vi "Test U8 Change FIFO Size.vi"() -> ()   [LabVIEW 2021]
uses:
  ChannelCommon/typedef/Direction.ctl
  ChannelCommon/typedef/TimeStamps.ctl
  CIF_Iceoryx_PCAP_Universal.lvclass
  D:/dev/Packages/CIF_Channels_Core/src/Iceorxy_Channels/CIF_Iceoryx_Chan/CIF_Iceoryx_Chn.lvclass
  ChannelCommon/typedef/New FIFO Instance Configuration.ctl
  Iceorxy Utilities/Typedef/PCAP Config.ctl
  ChannelCommon/typedef/New FIFO Config.ctl
  ChannelCommon/typedef/FIFO Flags.ctl
  Iceorxy Utilities/Typedef/PCAP Linktype.ctl
  CIF_Iceoryx_Chan/CIF_Iceoryx_Chn.lvclass
  ChannelCommon/ChannelCommon.lvlib
  Iceorxy Utilities/Iceoryx Channel Utilities.lvlib
panel:
  out "status":string
  out "pass":bool
  out "error out":errorcluster
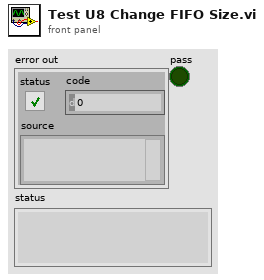
[diagram p1: front panel]
types:
  T1 = typedef "ChannelCommon.lvlib/Direction.ctl" = enum8{"Publisher", "Subscriber"}
  T2 = typedef "Iceoryx Channel Utilities.lvlib/PCAP Config.ctl" = cluster{"New FIFO Config":T3, "Linktype":T5, "Linktype Override":u32, "Type Name Override":string}
  T3 = typedef "ChannelCommon.lvlib/New FIFO Config.ctl" = cluster{"Max Bytes/Msg":u64, "Max Msg/FIFO":u64, "FIFO Flags":T4, "Best Effort Subscribers":u32, "Backpressure Subscribers":u32}
  T4 = typedef "ChannelCommon.lvlib/FIFO Flags.ctl" = cluster{"Backpressure":bool, "Extended Config":bool}
  T5 = typedef "Iceoryx Channel Utilities.lvlib/PCAP Linktype.ctl" = u32
  T6 = typedef "ChannelCommon.lvlib/New FIFO Instance Configuration.ctl" = cluster{"Backpressure":bool, "Bytes/Message Override":u32, "Messages/FIFO Override":u32, "Custom Data":u8[]}
  T7 = typedef "ChannelCommon.lvlib/TimeStamps.ctl" = cluster{"ClockID":u8, "T0":i64, "T_Out":i64}
  T8 = typedef "ChannelCommon.lvlib/New FIFO Instance Response.ctl" = cluster{"Publisher":string, "Custom Data":u8[]}
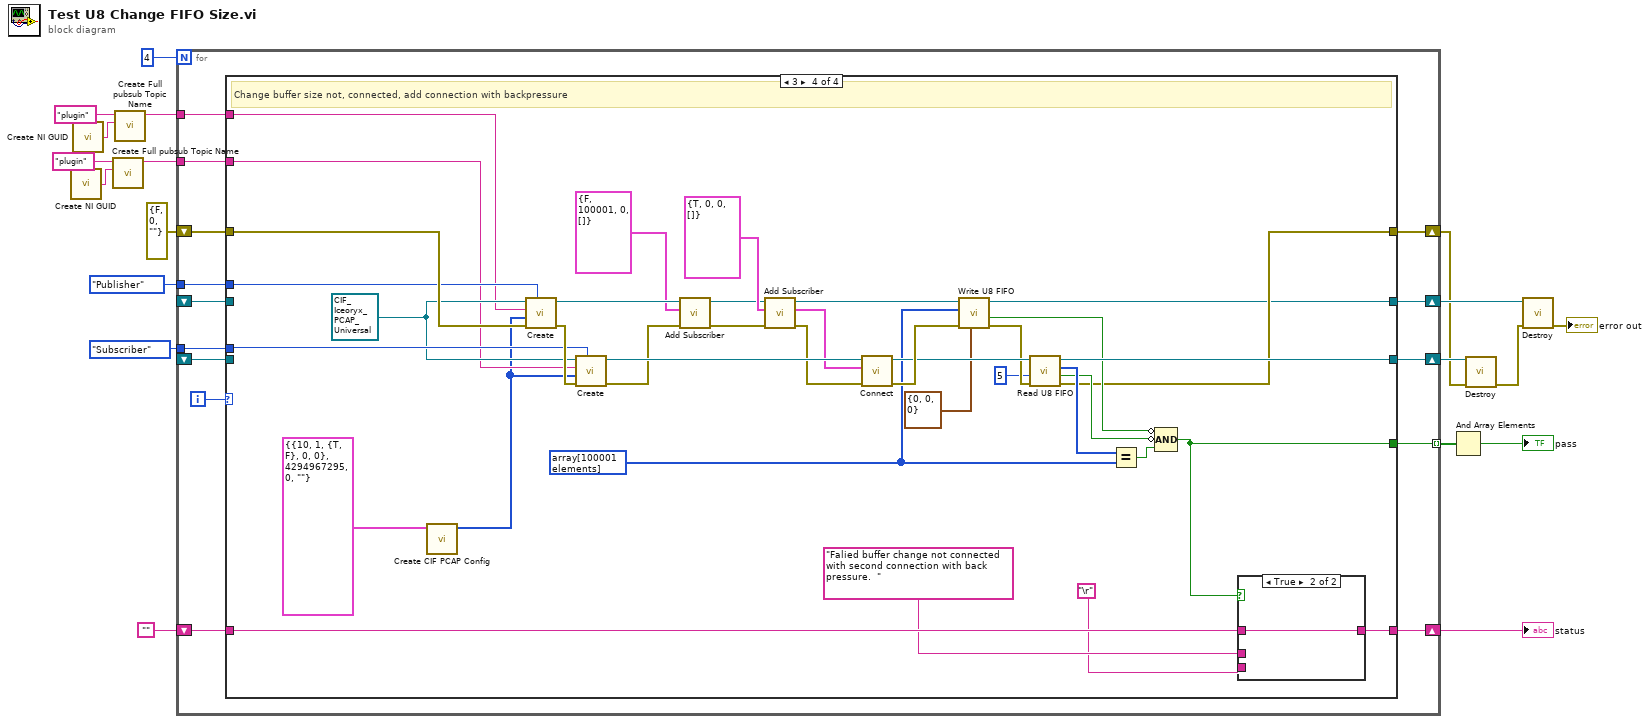
[diagram p0: block diagram]
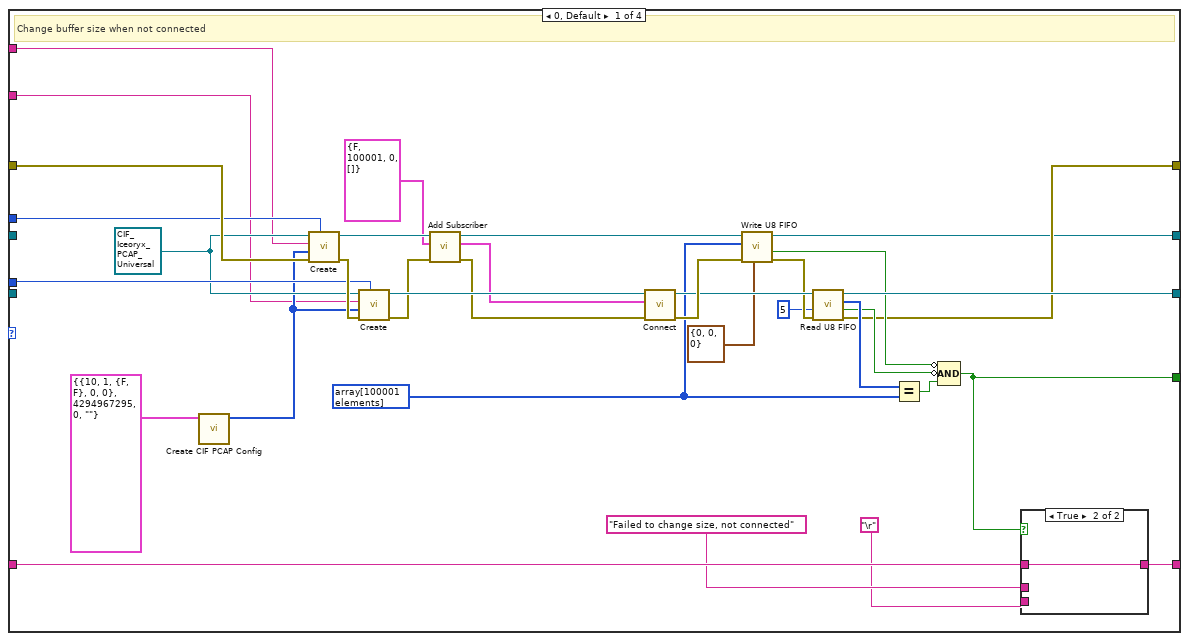
[diagram p2: hidden frame]
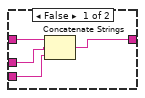
[diagram p3: hidden frame]
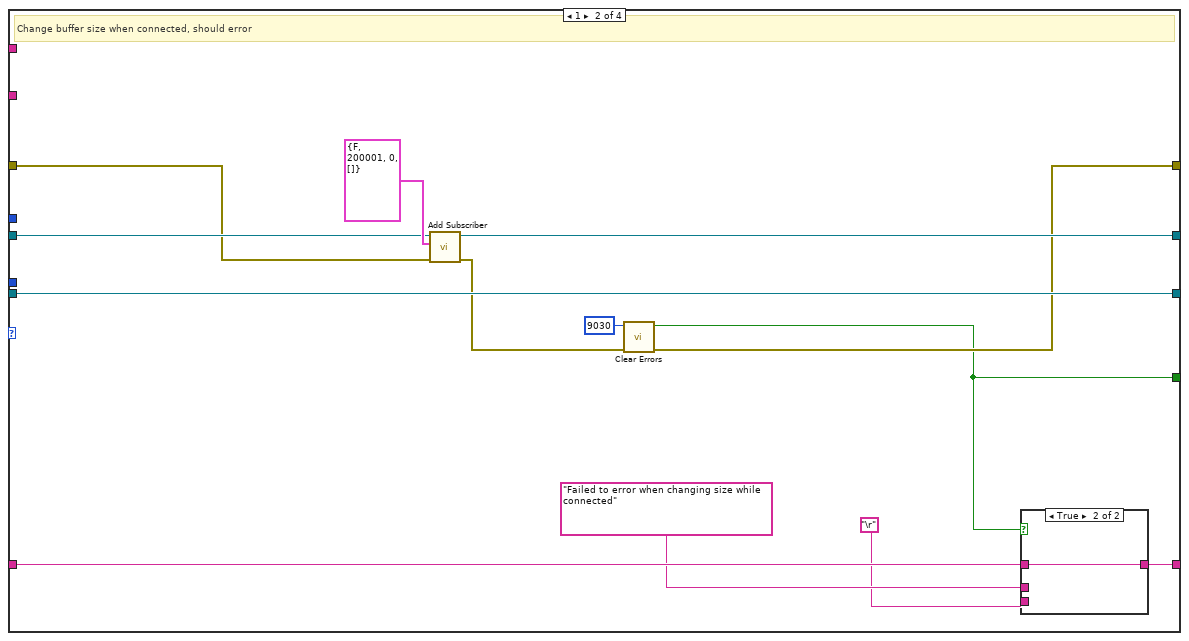
[diagram p4: hidden frame]
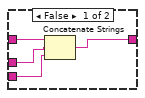
[diagram p5: hidden frame]
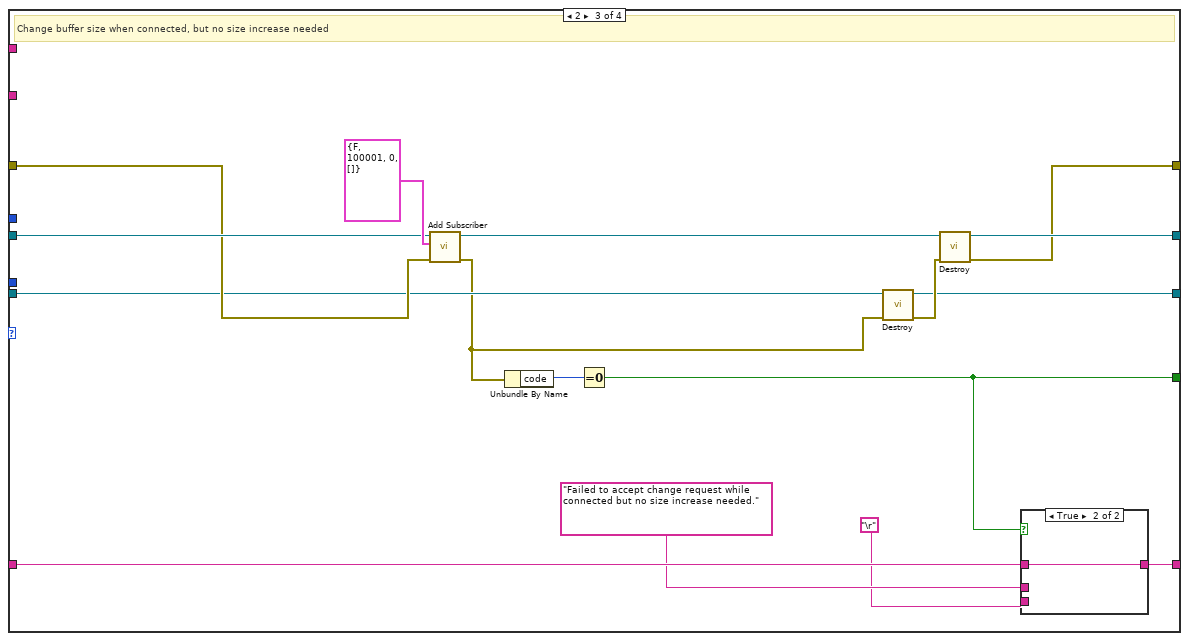
[diagram p6: hidden frame]
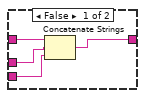
[diagram p7: hidden frame]
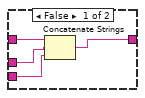
[diagram p8: hidden frame]
diagram:
  n1 = call <vilib>:"Create NI GUID.vi"() -> ("NI GUID"=w6:string)
  n2 = call <vilib>:"Create NI GUID.vi"() -> ("NI GUID"=w5:string)
  n3 = call "Create Full pubsub Topic Name.vi"("Topic"=w6, "Plugin name"="plugin") -> ("Full Topic"=w2:string)  [unwired: 8 in, 1 out]
  n4 = call "Create Full pubsub Topic Name.vi"("Topic"=w5, "Plugin name"="plugin") -> ("Full Topic"=w1:string)  [unwired: 8 in, 1 out]
  n5 = for {
    N: 4 -> [_]
    tunnel: [w33] -> w19 mode=indexing
    shift-right: [w31] -> w8
    shift-left: errorcluster {"status"=FALSE, "code"=0, "source"=""} ("error out") -> [w32]
    shift-right: [w28] -> w15
    shift-left: "" -> [w29]
    tunnel: Direction."Subscriber" ("Direction") -> [w27]
    tunnel: Direction."Publisher" ("Direction") -> [w26]
    shift-right: [w25] -> w11
    shift-left: _ -> [w23]
    shift-right: [w24] -> w10
    shift-left: _ -> [w22]
    tunnel: w2 -> [w21]
    tunnel: w1 -> [w20]
    i -> [w30]
    n6 = case shown="3" w30 {
      tunnel: [w62 w73 w98 w143] -> w33
      tunnel: w32 -> [w60 w79 w100 w141]
      tunnel: [w45 w75 w91 w126] -> w31
      tunnel: w29 -> [w67 w85 w106 w148]
      tunnel: [w66 w84 w105 w147] -> w28
      tunnel: w27 -> [w59 _ _ w140]
      tunnel: w26 -> [w58 _ _ w139]
      tunnel: [w54 w78 w92 w135] -> w25
      tunnel: [w44 w77 w93 w125] -> w24
      tunnel: w22 -> [_ w80 w101 _]
      tunnel: w23 -> [_ w78 w96 _]
      tunnel: w21 -> [w35 _ _ w114]
      tunnel: w20 -> [w34 _ _ w115]
      frame 0, Default {
        w49 = refnum<class "CIF_Iceoryx_PCAP_Universal.lvclass"> refnum ("CIF_CIPC_Fifo_U8.lvclass")
        w46 = u8[] array[100001 elements] ("U8 Data")
        # "Change buffer size when not connected"
        n7 = call "Create CIF PCAP Config.vi"("PCAP FIFO Config"=T2 {"New FIFO Config"={"Max Bytes/Msg"=10, "Max Msg/FIFO"=1, "FIFO Flags"={"Backpressure"=FALSE, "Extended Config"=FALSE}, "Best Effort Subscribers"=0, "Backpressure Subscribers"=0}, "Linktype"=4294967295, "Linktype Override"=0, "Type Name Override"=""}) -> ("Flattened PCAP FIFO Config"=w36:u8[])  [unwired: 10 in]
        n8 = call-dynamic "Create.vi"("Direction"=w58, "error in (no error)"=w60, "Custom Config Data"=w36, "Name"=w34, "CIFFIFO in"=w49) -> ("error out"=w61:errorcluster, "CIFFIFO out"=w43:refnum<class "CIF_Iceoryx_PCAP_Universal.lvclass">)  [unwired: 5 in]
        n9 = call-dynamic "Create.vi"("Direction"=w59, "error in (no error)"=w61, "Custom Config Data"=w36, "Name"=w35, "CIFFIFO in"=w49) -> ("error out"=w39:errorcluster, "CIFFIFO out"=w57:refnum<class "CIF_Iceoryx_PCAP_Universal.lvclass">)  [unwired: 5 in]
        n10 = call-dynamic "Add Subscriber.vi"("error in (no error)"=w39, "New FIFO Instance Config"=T6 {"Backpressure"=FALSE, "Bytes/Message Override"=100001, "Messages/FIFO Override"=0, "Custom Data"=[]}, "CIF_CIPC_Chn in"=w43) -> ("error out"=w38:errorcluster, "New FIFO Instance"=w41:T8, "CIF_CIPC_Chn out"=w42:refnum<class "CIF_Iceoryx_PCAP_Universal.lvclass">)  [unwired: 6 in]
        n11 = call-dynamic "Connect.vi"("error in (no error)"=w38, "Connection"=w41, "CIF_Iceoryx_PCAP"=w57) -> ("error out"=w56:errorcluster, "CIF_Iceoryx_PCAP"=w55:refnum<class "CIF_Iceoryx_PCAP_Universal.lvclass">)  [unwired: 7 in]
        n12 = call-dynamic "Write U8 FIFO.vi"("FIFO Timestamps"=T7 {"ClockID"=0, "T0"=0, "T_Out"=0}, "error in (no error)"=w56, "Data in"=w46, "CIFFIFO in"=w42) -> ("error out"=w53:errorcluster, "timed out?"=w52:bool, "CIFFIFO out"=w44:refnum<class "CIF_Iceoryx_PCAP_Universal.lvclass">)  [unwired: 4 in, 1 out]
        n13 = call-dynamic "Read U8 FIFO.vi"("error in (no error)"=w53, "Timeout (ms)"=5, "CIFFIFO in"=w55) -> ("error out"=w45:errorcluster, "timed out?"=w50:bool, "Data out"=w51:u8[], "CIFFIFO out"=w54:refnum<class "CIF_Iceoryx_PCAP_Universal.lvclass">)  [unwired: 4 in, 1 out]
        n14 = Equal?(x=w51, y=w46) -> (x = y?=w63:bool)
        n15 = Compound Arithmetic op=AND(invert w52, invert w50, w63) -> (w62:bool)
        n16 = case shown="True" w62 {
          tunnel: w67 -> [w71 w72]
          tunnel: [w68 w72] -> w66
          tunnel: "Failed to change size, not connected" -> [w70 _]
          tunnel: "\r" -> [w69 _]
          frame False {
            n17 = Concatenate Strings(w71, w70, w69) -> (w68:string)
          }
          frame True {
          }
        }
      }
      frame 1 {
        # "Change buffer size when connected, should error"
        n18 = call-dynamic "Add Subscriber.vi"("error in (no error)"=w79, "New FIFO Instance Config"=T6 {"Backpressure"=FALSE, "Bytes/Message Override"=200001, "Messages/FIFO Override"=0, "Custom Data"=[]}, "CIF_CIPC_Chn in"=w80) -> ("error out"=w76:errorcluster, "CIF_CIPC_Chn out"=w77:refnum<class "CIF_Iceoryx_Chn.lvclass">)  [unwired: 6 in, 1 out]
        n19 = call <vilib>:"Clear Errors.vi"("error in (no error)"=w76, "specific error code to clear (0: all)"=9030) -> ("error out"=w75:errorcluster, "specific error cleared?"=w73:bool)  [unwired: 4 in]
        n20 = case shown="True" w73 {
          tunnel: w85 -> [w89 w90]
          tunnel: [w86 w90] -> w84
          tunnel: "Failed to error when changing size while connected" -> [w88 _]
          tunnel: "\r" -> [w87 _]
          frame False {
            n21 = Concatenate Strings(w89, w88, w87) -> (w86:string)
          }
          frame True {
          }
        }
      }
      frame 2 {
        # "Change buffer size when connected, but no size increase needed"
        n22 = call-dynamic "Add Subscriber.vi"("error in (no error)"=w100, "New FIFO Instance Config"=T6 {"Backpressure"=FALSE, "Bytes/Message Override"=100001, "Messages/FIFO Override"=0, "Custom Data"=[]}, "CIF_CIPC_Chn in"=w101) -> ("error out"=w94:errorcluster, "CIF_CIPC_Chn out"=w95:refnum<class "CIF_Iceoryx_Chn.lvclass">)  [unwired: 6 in, 1 out]
        n23 = Unbundle By Name(w94) -> ("code"=w99:i32)
        n24 = Equal To 0?(x=w99) -> (x = 0?=w98:bool)
        n25 = call-dynamic "Destroy.vi"("error in (no error)"=w94, "CIFChannels in"=w96) -> ("error out"=w97:errorcluster, "CIFChannels out"=w92:refnum<class "CIF_Iceoryx_Chn.lvclass">)  [unwired: 8 in]
        n26 = call-dynamic "Destroy.vi"("error in (no error)"=w97, "CIFChannels in"=w95) -> ("error out"=w91:errorcluster, "CIFChannels out"=w93:refnum<class "CIF_Iceoryx_Chn.lvclass">)  [unwired: 8 in]
        n27 = case shown="True" w98 {
          tunnel: w106 -> [w110 w111]
          tunnel: [w107 w111] -> w105
          tunnel: "Failed to accept change request while connected but no size increase needed." -> [w109 _]
          tunnel: "\r" -> [w108 _]
          frame False {
            n28 = Concatenate Strings(w110, w109, w108) -> (w107:string)
          }
          frame True {
          }
        }
      }
      frame 3 {
        w130 = refnum<class "CIF_Iceoryx_PCAP_Universal.lvclass"> refnum ("CIF_CIPC_Fifo_U8.lvclass")
        w127 = u8[] array[100001 elements] ("U8 Data")
        # "Change buffer size not, connected, add connection with backpressure"
        n29 = call "Create CIF PCAP Config.vi"("PCAP FIFO Config"=T2 {"New FIFO Config"={"Max Bytes/Msg"=10, "Max Msg/FIFO"=1, "FIFO Flags"={"Backpressure"=TRUE, "Extended Config"=FALSE}, "Best Effort Subscribers"=0, "Backpressure Subscribers"=0}, "Linktype"=4294967295, "Linktype Override"=0, "Type Name Override"=""}) -> ("Flattened PCAP FIFO Config"=w112:u8[])  [unwired: 10 in]
        n30 = call-dynamic "Create.vi"("Direction"=w139, "error in (no error)"=w141, "Custom Config Data"=w112, "Name"=w115, "CIFFIFO in"=w130) -> ("error out"=w142:errorcluster, "CIFFIFO out"=w120:refnum<class "CIF_Iceoryx_PCAP_Universal.lvclass">)  [unwired: 5 in]
        n31 = call-dynamic "Create.vi"("Direction"=w140, "error in (no error)"=w142, "Custom Config Data"=w112, "Name"=w114, "CIFFIFO in"=w130) -> ("error out"=w117:errorcluster, "CIFFIFO out"=w138:refnum<class "CIF_Iceoryx_PCAP_Universal.lvclass">)  [unwired: 5 in]
        n32 = call-dynamic "Add Subscriber.vi"("error in (no error)"=w117, "New FIFO Instance Config"=T6 {"Backpressure"=FALSE, "Bytes/Message Override"=100001, "Messages/FIFO Override"=0, "Custom Data"=[]}, "CIF_CIPC_Chn in"=w120) -> ("error out"=w118:errorcluster, "CIF_CIPC_Chn out"=w119:refnum<class "CIF_Iceoryx_PCAP_Universal.lvclass">)  [unwired: 6 in, 1 out]
        n33 = call-dynamic "Add Subscriber.vi"("error in (no error)"=w118, "New FIFO Instance Config"=T6 {"Backpressure"=TRUE, "Bytes/Message Override"=0, "Messages/FIFO Override"=0, "Custom Data"=[]}, "CIF_CIPC_Chn in"=w119) -> ("error out"=w121:errorcluster, "New FIFO Instance"=w123:T8, "CIF_CIPC_Chn out"=w124:refnum<class "CIF_Iceoryx_PCAP_Universal.lvclass">)  [unwired: 6 in]
        n34 = call-dynamic "Connect.vi"("error in (no error)"=w121, "Connection"=w123, "CIF_Iceoryx_PCAP"=w138) -> ("error out"=w137:errorcluster, "CIF_Iceoryx_PCAP"=w136:refnum<class "CIF_Iceoryx_PCAP_Universal.lvclass">)  [unwired: 7 in]
        n35 = call-dynamic "Write U8 FIFO.vi"("FIFO Timestamps"=T7 {"ClockID"=0, "T0"=0, "T_Out"=0}, "error in (no error)"=w137, "Data in"=w127, "CIFFIFO in"=w124) -> ("error out"=w134:errorcluster, "timed out?"=w133:bool, "CIFFIFO out"=w125:refnum<class "CIF_Iceoryx_PCAP_Universal.lvclass">)  [unwired: 4 in, 1 out]
        n36 = call-dynamic "Read U8 FIFO.vi"("error in (no error)"=w134, "Timeout (ms)"=5, "CIFFIFO in"=w136) -> ("error out"=w126:errorcluster, "timed out?"=w131:bool, "Data out"=w132:u8[], "CIFFIFO out"=w135:refnum<class "CIF_Iceoryx_PCAP_Universal.lvclass">)  [unwired: 4 in, 1 out]
        n37 = Equal?(x=w132, y=w127) -> (x = y?=w144:bool)
        n38 = Compound Arithmetic op=AND(invert w133, invert w131, w144) -> (w143:bool)
        n39 = case shown="True" w143 {
          tunnel: w148 -> [w152 w153]
          tunnel: [w149 w153] -> w147
          tunnel: "Falied buffer change not connected with second connection with back pressure.  " -> [w151 _]
          tunnel: "\r" -> [w150 _]
          frame False {
            n40 = Concatenate Strings(w152, w151, w150) -> (w149:string)
          }
          frame True {
          }
        }
      }
    }
  }
  "status" <- w15
  n41 = And Array Elements(Boolean array=w19) -> (logical AND=→"pass":bool)
  n42 = call-dynamic "Destroy.vi"("error in (no error)"=w8, "CIFChannels in"=w11) -> ("error out"=w9:errorcluster)  [unwired: 8 in, 1 out]
  n43 = call-dynamic "Destroy.vi"("error in (no error)"=w9, "CIFChannels in"=w10) -> ("error out"=→"error out":errorcluster)  [unwired: 8 in, 1 out]
